vi "CO move TurnTable.vi"(8 "error in (no error)":errorcluster caption="에러 입력(에러 없음)", 10 "Turn Table Info":T1, 11 "Instrument Manager 입력":refnum<class "Instrument Manager.lvclass">) -> (0 "error out":errorcluster caption="에러 출력", 3 "Instrument Manager 출력":refnum<class "Instrument Manager.lvclass">)   [LabVIEW 2023, in "Instrument Manager.lvclass"]
uses:
  Instrument Manager.lvclass
  Instrument Manager.lvclass/Instrument Manager.ctl
  Module/Turn Table and Mast Control/Interface Class/Turn Table/Interface - Turn Table.lvclass
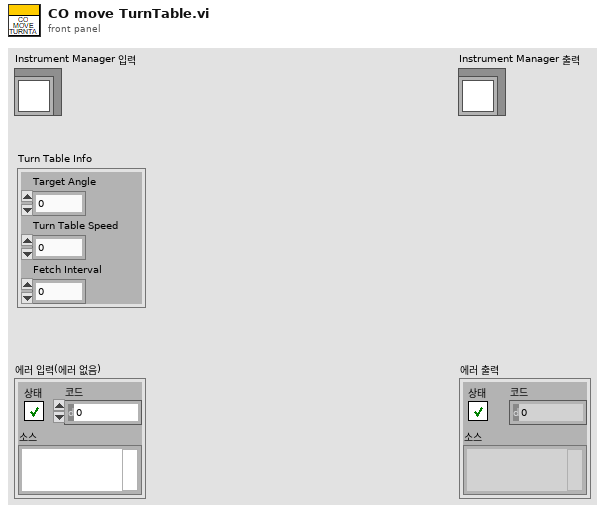
[diagram p1: front panel]
types:
  T1 = cluster{"Target Angle":dbl, "Turn Table Speed":i32, "Fetch Interval":i32}
  T2 = cluster{"Anritsu Call Box":refnum<class "Anritsu Call Box.lvclass">, "Spectrum Analyzer":refnum<class "Interface_Spectrum.lvclass">, "RF Switch Box":refnum<class "RF Filter Box.lvclass">, "Turn Table":refnum<class "Interface - Turn Table.lvclass">, "Mast":refnum<class "Interface - Mast.lvclass">, "3D Controller":refnum<class "Interface_3D Controller.lvclass">}
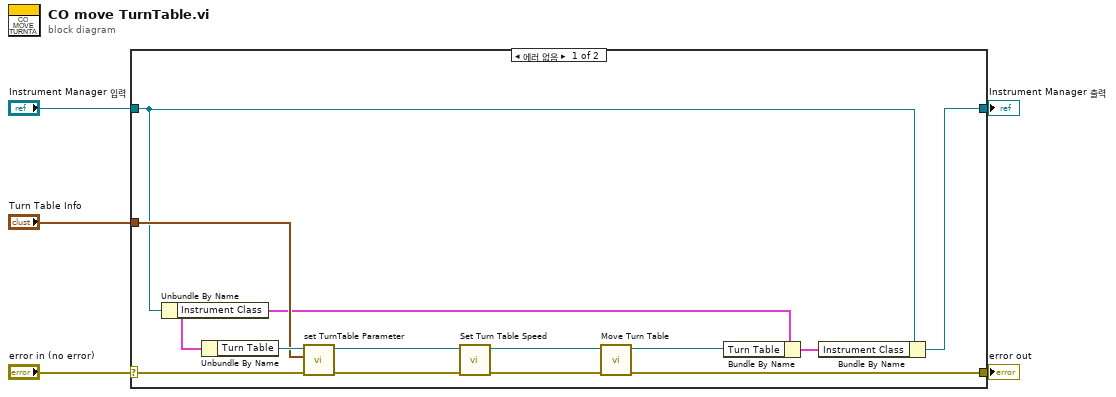
[diagram p0: block diagram]
diagram:
  n1 = case shown="에러 없음" "error in (no error)" {
    selector: "error in (no error)" -> [w18 w20]
    tunnel: [w15 w20] -> w4
    tunnel: [w6 w19] -> w2
    tunnel: "Instrument Manager 입력" -> [w8 w19]
    tunnel: "Turn Table Info" -> [w13 _]
    frame No Error {
      n2 = Unbundle By Name(w8) -> ("Instrument Class"=w10:T2)
      n3 = Unbundle By Name(w10) -> ("Turn Table"=w14:refnum<class "Interface - Turn Table.lvclass">)
      n4 = call-dynamic "set TurnTable Parameter.vi"("error in (no error)"=w18, "Turn Table Info"=w13, "Interface - Turn Table in"=w14) -> ("error out"=w17:errorcluster, "Interface - Turn Table out"=w12:refnum<class "Interface - Turn Table.lvclass">)  [unwired: 7 in]
      n5 = call-dynamic "Set Turn Table Speed.vi"("error in (no error)"=w17, "Interface - Turn Table in"=w12) -> ("error out"=w16:errorcluster, "Interface - Turn Table out"=w11:refnum<class "Interface - Turn Table.lvclass">)  [unwired: 8 in]
      n6 = call-dynamic "Move Turn Table.vi"("error in (no error)"=w16, "Interface - Turn Table in"=w11) -> ("error out"=w15:errorcluster, "Interface - Turn Table out"=w9:refnum<class "Interface - Turn Table.lvclass">)  [unwired: 8 in]
      n7 = Bundle By Name(cluster=w10, "Turn Table"=w9) -> (w7:T2)
      n8 = Bundle By Name(cluster=w8, "Instrument Class"=w7) -> (w6:refnum<class "Instrument Manager.lvclass">)
    }
    frame Error {
    }
  }
  "error out" <- w4
  "Instrument Manager 출력" <- w2
